vi "Append New Page.vi"(6 "Set as active (T)":bool=TRUE, 8 "error in (no error)":errorcluster, 10 "Page Name":string, 11 "Document in":refnum<class "Document.lvclass">) -> (0 "error out":errorcluster, 1 "Created?":bool, 2 "Created Page Name":string, 3 "Document out":refnum<class "Document.lvclass">)   [LabVIEW 2017, in "LabVIEW NPOI.lvlib" / "Document.lvclass"]
doc: "Create new page to the <b>Document</b>, nammed <b>Page Name</b>."
uses:
  Document.lvclass
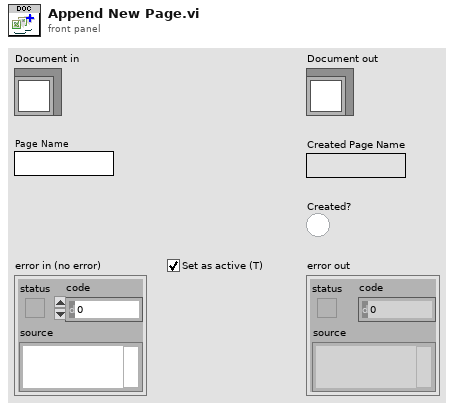
[diagram p1: front panel]
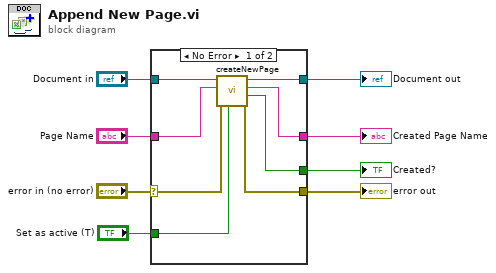
[diagram p0: block diagram]
diagram:
  n1 = case shown="No Error" "error in (no error)" {
    selector: "error in (no error)" -> [w13 w17]
    tunnel: "Document in" -> [w16 w18]
    tunnel: [w15 w18] -> w7
    tunnel: [w12 w17] -> w5
    tunnel: "Page Name" -> [w14 _]
    tunnel: "Set as active (T)" -> [w9 _]
    tunnel: [w11 _] -> w2
    tunnel: [w10 _] -> w1
    frame No Error {
      n2 = call-dynamic "createNewPage.vi"("Set as active (T)"=w9, "error in (no error)"=w13, "Page Name"=w14, "Document in"=w16) -> ("error out"=w12:errorcluster, "Created?"=w10:bool, "Created Page Name"=w11:string, "Document out"=w15:refnum<class "Document.lvclass">)  [unwired: 4 in]
    }
    frame Error {
    }
  }
  "error out" <- w5
  "Document out" <- w7
  "Created?" <- w1
  "Created Page Name" <- w2
